vi "edge_finder_3.vi"(0 "right_edge_location":cluster{"X":sgl, "Y":sgl}[](array[cluster]), 1 "mid_edge_location":cluster{"X":sgl, "Y":sgl}[](array[cluster]), 5 "left_edge_location":cluster{"X":sgl, "Y":sgl}[](array[cluster]), 7 "Mid_center in":dbl, 9 "Left_center in":dbl, 12 "Right_center in":dbl, 13 "Reset_ROI":dbl) -> (2 "mid_roi_dead":bool, 3 "left_line_center":dbl, 4 "right_line_center":dbl, 6 "left_roi_dead":bool, 8 "right_roi_dead":bool, 10 "mid_center out":dbl, 14 "mid_roi_dead":bool)   [LabVIEW 2024]
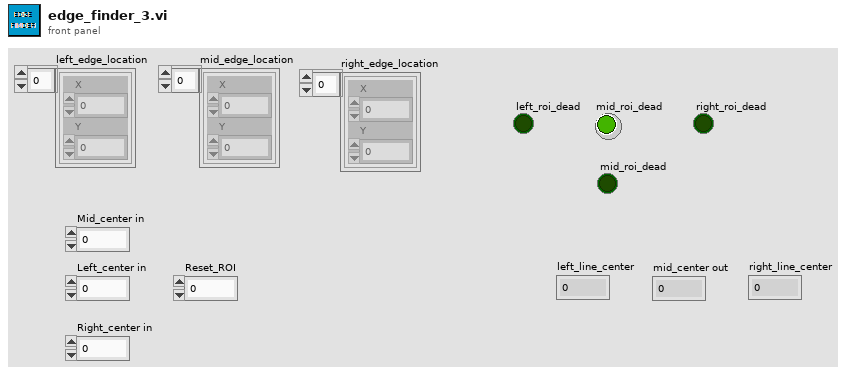
[diagram p1: front panel]
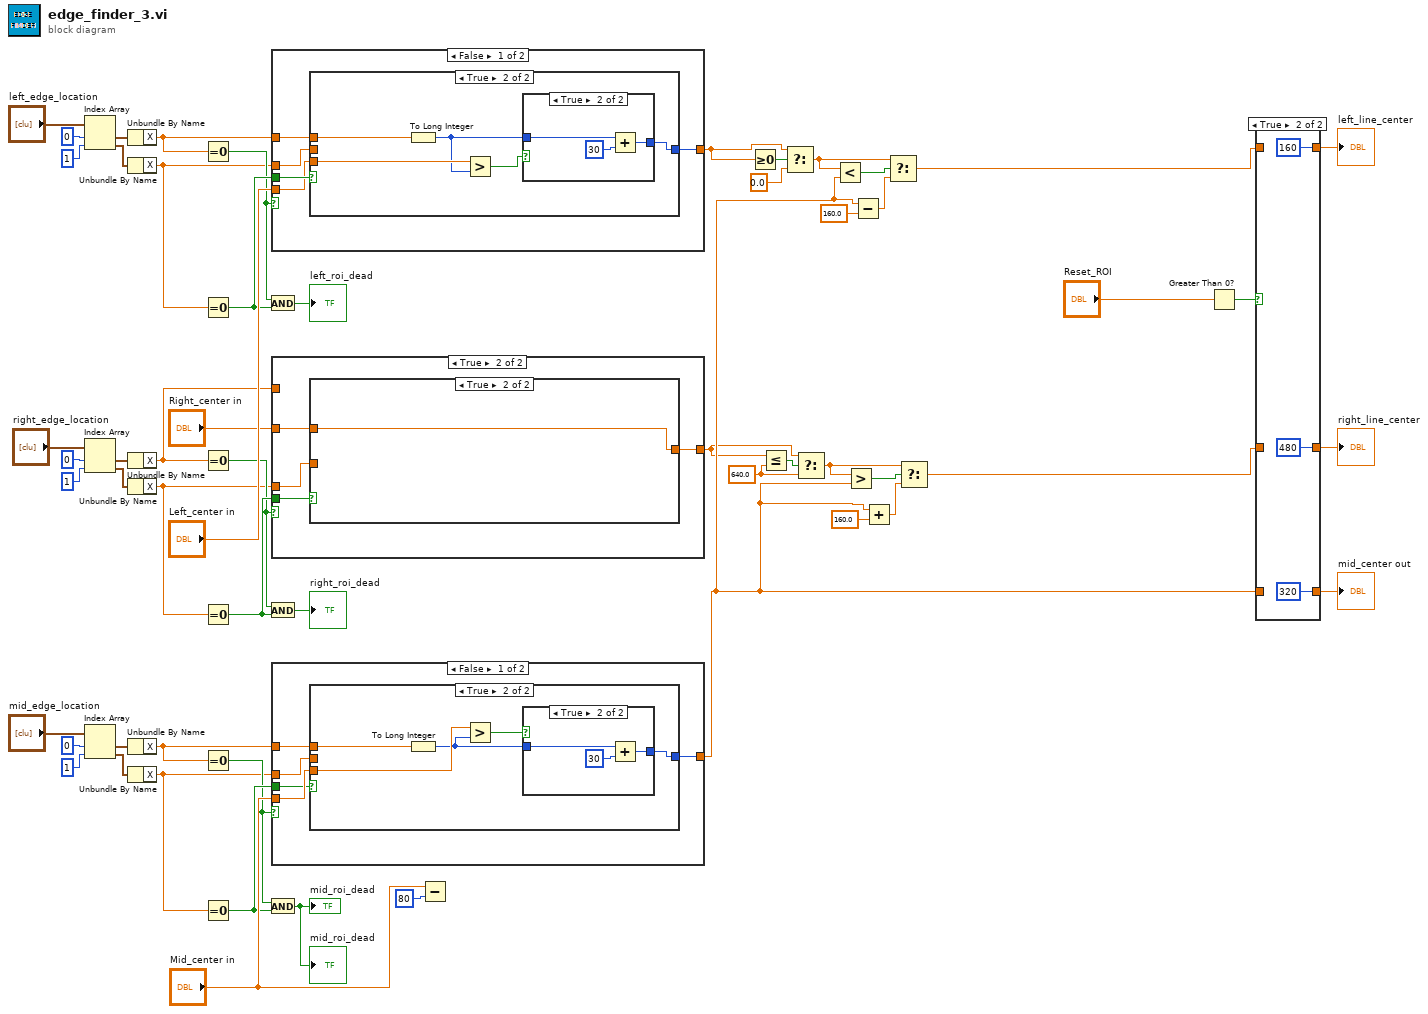
[diagram p0: block diagram]
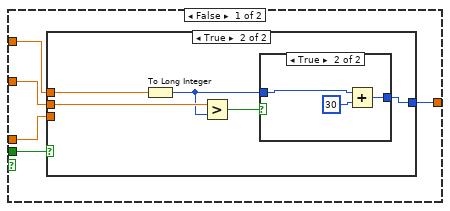
[diagram p3: hidden frame]
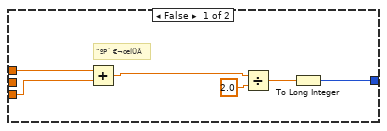
[diagram p4: hidden frame]
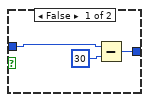
[diagram p5: hidden frame]
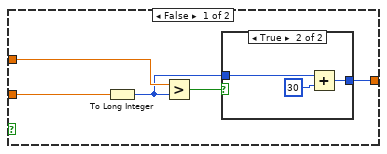
[diagram p6: hidden frame]
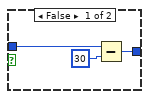
[diagram p7: hidden frame]
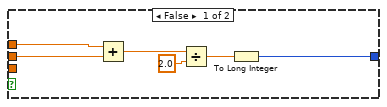
[diagram p8: hidden frame]
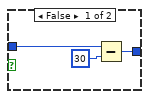
[diagram p9: hidden frame]
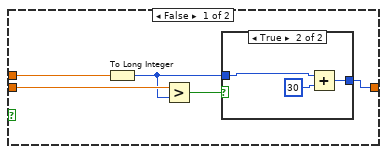
[diagram p11: hidden frame]
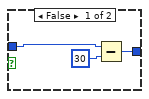
[diagram p12: hidden frame]
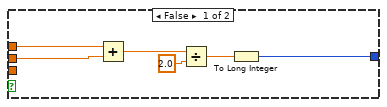
[diagram p13: hidden frame]
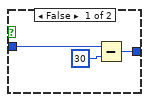
[diagram p14: hidden frame]
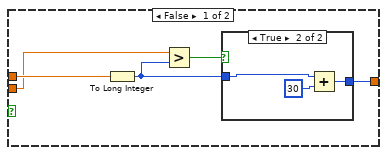
[diagram p16: hidden frame]
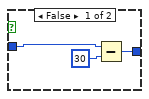
[diagram p17: hidden frame]
diagram:
  w8 = 640.0 ("y")
  n1 = Index Array(array="left_edge_location", index #1=0 ("인덱스"), index #2=1 ("인덱스")) -> (element #1=w32:cluster{"X":sgl, "Y":sgl}, element #2=w33:cluster{"X":sgl, "Y":sgl})
  n2 = Index Array(array="right_edge_location", index #1=0 ("인덱스"), index #2=1 ("인덱스")) -> (element #1=w34:cluster{"X":sgl, "Y":sgl}, element #2=w35:cluster{"X":sgl, "Y":sgl})
  n3 = Index Array(array="mid_edge_location", index #1=0 ("인덱스"), index #2=1 ("인덱스")) -> (element #1=w22:cluster{"X":sgl, "Y":sgl}, element #2=w23:cluster{"X":sgl, "Y":sgl})
  n4 = Unbundle By Name(w32) -> ("X"=w38:sgl)
  n5 = Unbundle By Name(w33) -> ("X"=w39:sgl)
  n6 = Unbundle By Name(w34) -> ("X"=w37:sgl)
  n7 = Unbundle By Name(w35) -> ("X"=w36:sgl)
  n8 = Unbundle By Name(w22) -> ("X"=w24:sgl)
  n9 = Unbundle By Name(w23) -> ("X"=w25:sgl)
  n10 = Equal To 0?(x=w38) -> (x = 0?=w40:bool)
  n11 = Equal To 0?(x=w39) -> (x = 0?=w41:bool)
  n12 = Equal To 0?(x=w37) -> (x = 0?=w42:bool)
  n13 = Equal To 0?(x=w36) -> (x = 0?=w43:bool)
  n14 = Equal To 0?(x=w24) -> (x = 0?=w26:bool)
  n15 = Equal To 0?(x=w25) -> (x = 0?=w27:bool)
  n16 = And(x=w40, y=w41) -> (x .and. y?=→"left_roi_dead":bool)
  n17 = And(x=w42, y=w43) -> (x .and. y?=→"right_roi_dead":bool)
  n18 = And(x=w26, y=w27) -> (x .and. y?=→"mid_roi_dead" →"mid_roi_dead":bool)
  n19 = case shown="False" w40 {
    tunnel: w41 -> [w61 w82]
    tunnel: w38 -> [w60 _]
    tunnel: w39 -> [w59 w79]
    tunnel: "Left_center in" -> [w57 w81]
    tunnel: [w58 w80] -> w7
    frame False {
      n20 = case shown="True" w61 {
        tunnel: w60 -> [w67 w70]
        tunnel: w59 -> [w66 _]
        tunnel: [w62 w68] -> w58
        tunnel: w57 -> [_ w72]
        frame False {
          n21 = Add(x=w67, y=w66) -> (x+y=w65:sgl)
          n22 = Divide(x=w65, y=sgl 2.0) -> (x/y=w63:sgl)
          n23 = To Long Integer(number=w63) -> (32bit integer=w62:i32)
        }
        frame True {
          n24 = To Long Integer(number=w70) -> (32bit integer=w69:i32)
          n25 = Greater?(x=w72, y=w69) -> (0:w71:bool)
          n26 = case shown="True" w71 {
            tunnel: w69 -> [w75 w78]
            tunnel: [w73 w76] -> w68
            frame False {
              n27 = Subtract(x=w75, y=30) -> (x-y=w73:i32)
            }
            frame True {
              n28 = Add(x=w78, y=30) -> (x+y=w76:i32)
            }
          }
        }
      }
    }
    frame True {
      n29 = case shown="True" w82 {
        tunnel: w81 -> [w87 w94]
        tunnel: [w83 w94] -> w80
        tunnel: w79 -> [w86 _]
        frame False {
          n30 = To Long Integer(number=w86) -> (32bit integer=w84:i32)
          n31 = Greater?(x=w87, y=w84) -> (0:w85:bool)
          n32 = case shown="True" w85 {
            tunnel: [w89 w92] -> w83
            tunnel: w84 -> [w88 w91]
            frame False {
              n33 = Subtract(x=w88, y=30) -> (x-y=w89:i32)
            }
            frame True {
              n34 = Add(x=w91, y=30) -> (x+y=w92:i32)
            }
          }
        }
        frame True {
        }
      }
    }
  }
  n35 = case shown="True" w42 {
    tunnel: w43 -> [w99 w120]
    tunnel: w37 -> [w98 _]
    tunnel: w36 -> [w97 w117]
    tunnel: "Right_center in" -> [w95 w119]
    tunnel: [w96 w118] -> w4
    frame False {
      n36 = case shown="True" w99 {
        tunnel: w98 -> [w105 w108]
        tunnel: w97 -> [w104 _]
        tunnel: [w100 w106] -> w96
        tunnel: w95 -> [_ w110]
        frame False {
          # "¨ºP´ €¬œÍÜÂ"
          n37 = Add(x=w105, y=w104) -> (x+y=w103:sgl)
          n38 = Divide(x=w103, y=sgl 2.0) -> (x/y=w101:sgl)
          n39 = To Long Integer(number=w101) -> (32bit integer=w100:i32)
        }
        frame True {
          n40 = To Long Integer(number=w108) -> (32bit integer=w107:i32)
          n41 = Greater?(x=w110, y=w107) -> (0:w109:bool)
          n42 = case shown="True" w109 {
            tunnel: w107 -> [w113 w116]
            tunnel: [w111 w114] -> w106
            frame False {
              n43 = Subtract(x=w113, y=30) -> (x-y=w111:i32)
            }
            frame True {
              n44 = Add(x=w116, y=30) -> (x+y=w114:i32)
            }
          }
        }
      }
    }
    frame True {
      n45 = case shown="True" w120 {
        tunnel: w119 -> [w125 w132]
        tunnel: [w121 w132] -> w118
        tunnel: w117 -> [w124 _]
        frame False {
          n46 = To Long Integer(number=w124) -> (32bit integer=w122:i32)
          n47 = Greater?(x=w125, y=w122) -> (0:w123:bool)
          n48 = case shown="True" w123 {
            tunnel: [w127 w130] -> w121
            tunnel: w122 -> [w126 w129]
            frame False {
              n49 = Subtract(x=w126, y=30) -> (x-y=w127:i32)
            }
            frame True {
              n50 = Add(x=w129, y=30) -> (x+y=w130:i32)
            }
          }
        }
        frame True {
        }
      }
    }
  }
  n51 = case shown="False" w26 {
    tunnel: w27 -> [w133 w158]
    tunnel: w24 -> [w136 _]
    tunnel: w25 -> [w135 w155]
    tunnel: "Mid_center in" -> [w137 w157]
    tunnel: [w134 w156] -> w12
    frame False {
      n52 = case shown="True" w133 {
        tunnel: w136 -> [w143 w146]
        tunnel: w135 -> [w142 _]
        tunnel: [w138 w144] -> w134
        tunnel: w137 -> [_ w148]
        frame False {
          n53 = Add(x=w143, y=w142) -> (x+y=w141:sgl)
          n54 = Divide(x=w141, y=sgl 2.0) -> (x/y=w139:sgl)
          n55 = To Long Integer(number=w139) -> (32bit integer=w138:i32)
        }
        frame True {
          n56 = To Long Integer(number=w146) -> (32bit integer=w145:i32)
          n57 = Greater?(x=w148, y=w145) -> (0:w147:bool)
          n58 = case shown="True" w147 {
            tunnel: w145 -> [w151 w154]
            tunnel: [w149 w152] -> w144
            frame False {
              n59 = Subtract(x=w151, y=30) -> (x-y=w149:i32)
            }
            frame True {
              n60 = Add(x=w154, y=30) -> (x+y=w152:i32)
            }
          }
        }
      }
    }
    frame True {
      n61 = case shown="True" w158 {
        tunnel: w157 -> [w162 w170]
        tunnel: [w159 w170] -> w156
        tunnel: w155 -> [w163 _]
        frame False {
          n62 = To Long Integer(number=w163) -> (32bit integer=w160:i32)
          n63 = Greater?(x=w162, y=w160) -> (0:w161:bool)
          n64 = case shown="True" w161 {
            tunnel: w160 -> [w165 w169]
            tunnel: [w164 w167] -> w159
            frame False {
              n65 = Subtract(x=w165, y=30) -> (x-y=w164:i32)
            }
            frame True {
              n66 = Add(x=w169, y=30) -> (x+y=w167:i32)
            }
          }
        }
        frame True {
        }
      }
    }
  }
  n67 = Subtract(x="Mid_center in", y=80) -> ()  [unwired: 1 out]
  n68 = Greater Or Equal To 0?(x=w7) -> (x >= 0?=w15:bool)
  n69 = Less Or Equal?(x=w4, y=w8) -> (x <= y?=w9:bool)
  n70 = Select(t=w7, s=w15, f=0.0) -> (s? t:f=w6:dbl)
  n71 = Select(t=w4, s=w9, f=w8) -> (s? t:f=w3:dbl)
  n72 = Less?(x=w6, y=w12) -> (x < y?=w18:bool)
  n73 = Greater?(x=w3, y=w12) -> (0:w13:bool)
  n74 = Subtract(x=w12, y=160.0) -> (x-y=w16:dbl)
  n75 = Add(x=w12, y=160.0) -> (x+y=w10:dbl)
  n76 = Select(t=w6, s=w18, f=w16) -> (s? t:f=w5:dbl)
  n77 = Select(t=w3, s=w13, f=w10) -> (s? t:f=w2:dbl)
  n78 = Greater Than 0?(x="Reset_ROI") -> (x > 0?=w56:bool)
  n79 = case shown="True" w56 {
    tunnel: w2 -> [w173 _]
    tunnel: [w173 480 ("상위 리미트")] -> w51
    tunnel: w5 -> [w172 _]
    tunnel: [w172 160 ("하위 리미트")] -> w50
    tunnel: w12 -> [w171 _]
    tunnel: [w171 320 ("하위 리미트")] -> w53
    frame False {
    }
    frame True {
    }
  }
  "mid_center out" <- w53
  "right_line_center" <- w51
  "left_line_center" <- w50
